vi "Destroy.vi"(8 "error in (no error)":errorcluster, 11 "object in":refnum<class "Channel.lvclass">) -> (0 "error out":errorcluster, 3 "object out":refnum<class "Channel.lvclass">)   [LabVIEW 2021, in "Channel.lvlib" / "Channel.lvclass"]
doc: "Releases all the references"
uses:
  Channel.lvclass
  Configuration_class/Configuration.lvclass
  Channel.lvclass/Channel.ctl
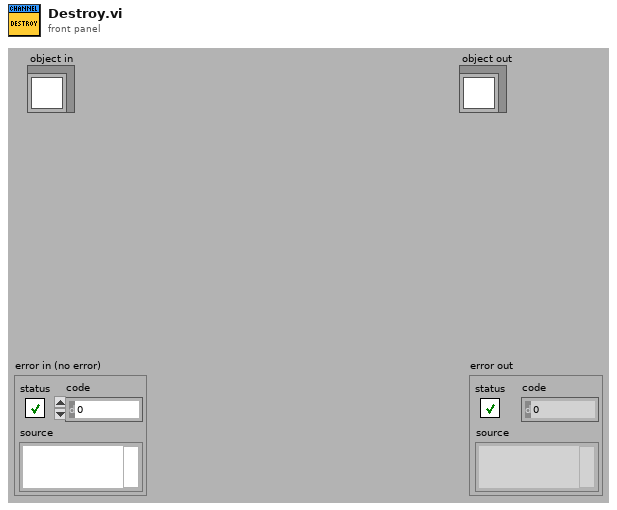
[diagram p1: front panel]
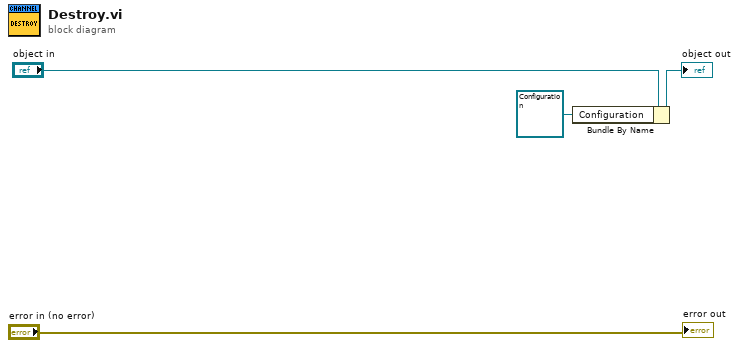
[diagram p0: block diagram]
diagram:
  n1 = Bundle By Name(cluster="object in", "Configuration"=refnum<class "Configuration.lvclass"> refnum) -> (→"object out":refnum<class "Channel.lvclass">)
  "error out" <- "error in (no error)"
